vi "Set Parent.vi"(8 "error in (no error)":errorcluster, 10 "Parent":refnum<data-value>, 11 "NodeRef In":refnum<data-value>) -> (0 "error out":errorcluster, 3 "NodeRef":refnum<data-value>)   [LabVIEW 2020, in "PicoG-ParserLexer.lvlib" / "Node.lvclass"]
doc: "Sets this node's parent if not already set. If this node already has a parent then RemoveChild must be called on the parent with this node first.\n\n<b>Error Codes:</b>\n<b>1556</b>: Node not instantiated with Ctor first, reference invalid.\n<b>14</b>: Parent is already assigned. Call RemoveChild on parent first."
uses:
  Node.lvclass
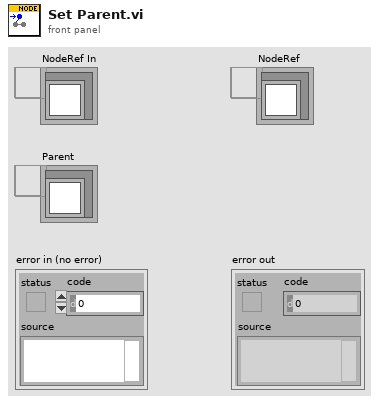
[diagram p1: front panel]
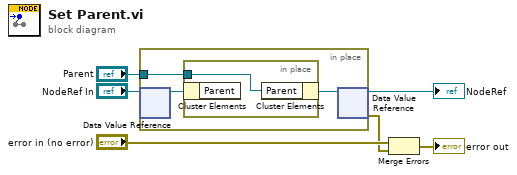
[diagram p0: block diagram]
diagram:
  n1 = in-place {
    in-place-border: "Parent" -> [w8]
    n2 = in-place-dvr #1("NodeRef In") -> (w9:refnum<class "Node.lvclass">)  [unwired: 1 out]
    n3 = in-place {
      in-place-border: w8 -> [w10]
      n4 = in-place-cluster #2(w9) -> ()  [unwired: 1 out]
      n5 = in-place-cluster #2("Parent"=w10) -> (w7:refnum<class "Node.lvclass">)
    }
    n6 = in-place-dvr #1(w7) -> (→"NodeRef":refnum<data-value>, w1:errorcluster)
  }
  n7 = Merge Errors("error in (no error)", w1) -> (→"error out":errorcluster)
